vi "Reset Fault.vi"(8 "error in (no error)":errorcluster, 11 "ServoDrive in":refnum<class "ServoDrive.lvclass">) -> (0 "error out":errorcluster, 3 "ServoDrive out":refnum<class "ServoDrive.lvclass">)   [LabVIEW 2021, in "ServoDrive.lvclass"]
uses:
  ServoDrive.lvclass
  ServoDrive.lvclass/ServoDrive.ctl
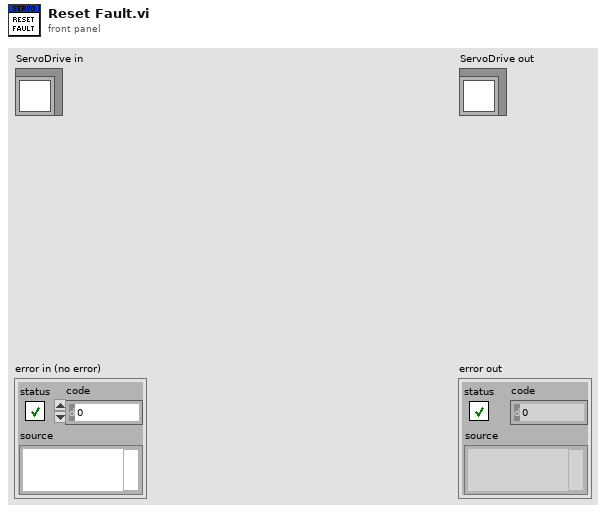
[diagram p1: front panel]
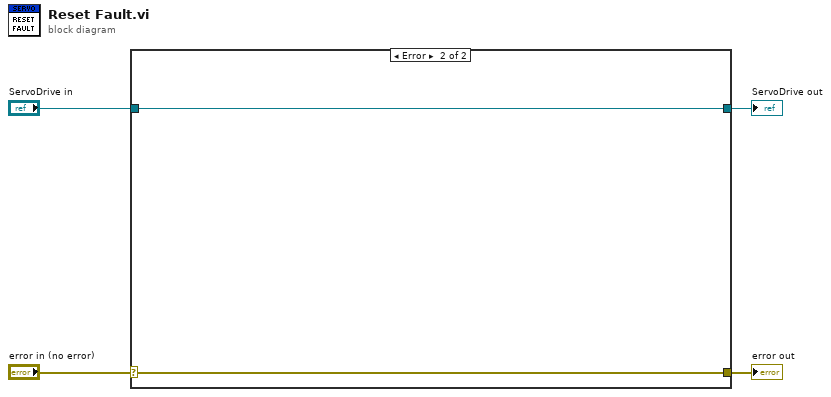
[diagram p0: block diagram]
diagram:
  n1 = case shown="Error" "error in (no error)" {
    selector: "error in (no error)" -> [w5 w8]
    tunnel: [w5 w8] -> w3
    tunnel: [w6 w7] -> w1
    tunnel: "ServoDrive in" -> [w6 w7]
    frame No Error {
      # "Wire the error cluster across even in the \"No Error\"\ncase so that warnings get propagated."
    }
    frame Error {
    }
  }
  "error out" <- w3
  "ServoDrive out" <- w1
